vi "str16tonum.vi"(11 "字符串":string) -> (3 "数值":i32)   [LabVIEW 2026, in "UI-距离测量.lvlib"]
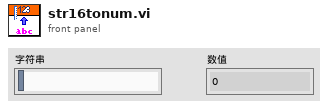
[diagram p1: front panel]
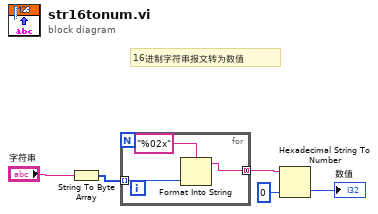
[diagram p0: block diagram]
diagram:
  # "16进制字符串报文转为数值"
  n1 = String To Byte Array(string="字符串") -> (unsigned byte array=w4:u8[])
  n2 = for {
    tunnel: w4 -> [w8] mode=indexing
    tunnel: [w6] -> w5 mode=concatenating
    n3 = Format Into String(format string="%02x" ("格式字符串"), w8) -> (resulting string=w6:string)  [unwired: 2 in, 1 out]
  }
  n4 = Hexadecimal String To Number(string=w5, default (0uL)=0 ("默认(0 U32)")) -> (number=→"数值":i32)  [unwired: 1 in, 1 out]
